vi "FRC Copy Files Recursive.vi"(0 "source project folder":path, 7 "target project folder":path, 11 "error in":errorcluster) -> (4 "target path out":path, 15 "error out":errorcluster)   [LabVIEW 2027]
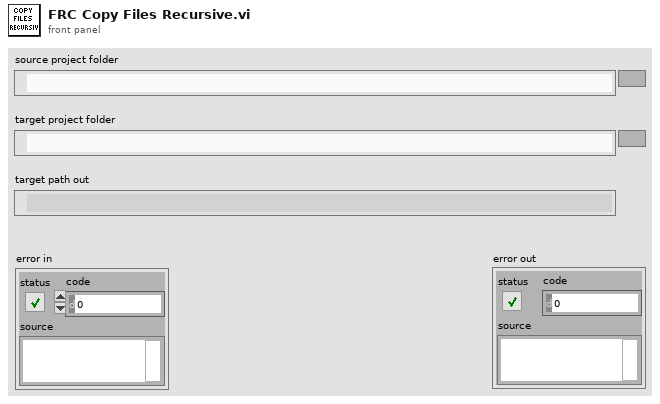
[diagram p1: front panel]
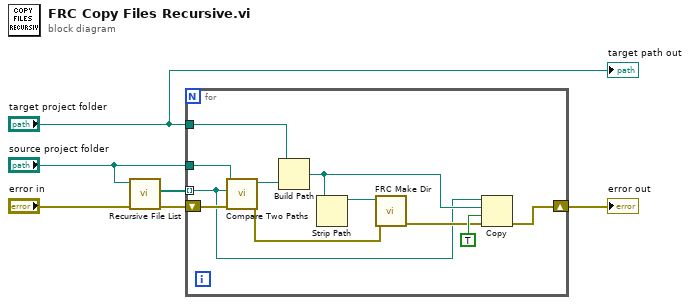
[diagram p0: block diagram]
diagram:
  n1 = call <vilib>:"Recursive File List.vi"("error in (no error)"="error in", "Folder Path"="source project folder") -> ("error out"=w4:errorcluster, "All Files in Dir"=w6:path[])  [unwired: 5 in, 3 out]
  n2 = for {
    tunnel: w6 -> [w8] mode=indexing
    tunnel: "source project folder" -> [w17]
    tunnel: "target project folder" -> [w15]
    shift-right: [w7] -> w3
    shift-left: w4 -> [w12]
    n3 = call <vilib>:"Compare Two Paths.vi"("error in (no error)"=w12, "Path 2"=w8, "Path 1"=w17) -> ("error out"=w11:errorcluster, "Relative Path from 1 to 2"=w16:path)  [unwired: 5 in, 2 out]
    n4 = Build Path(base path=w15, name or relative path=w16) -> (appended path=w9:path)
    n5 = Strip Path(path=w9) -> (stripped path=w14:path)  [unwired: 1 out]
    n6 = call <resource>:"FRC Make Dir.vi"("error in"=w11, "path"=w14) -> ("error out"=w10:errorcluster)  [unwired: 9 in]
    n7 = Copy(8:w10, 9:TRUE ("overwrite (F)"), 10:w9, 11:w8) -> (0:w7:errorcluster)  [unwired: 1 in, 2 out]
  }
  "error out" <- w3
  "target path out" <- "target project folder"
